vi "VIH UI - Project XML Indicator.vi"(11 "XML in":string) -> ()   [LabVIEW 2014]
doc: "::: VI Helpeks :::\nCopyright (c) 2000-2026 Konstantin Shifershteyn. All rights reserved."
panel:
  out "XML":string
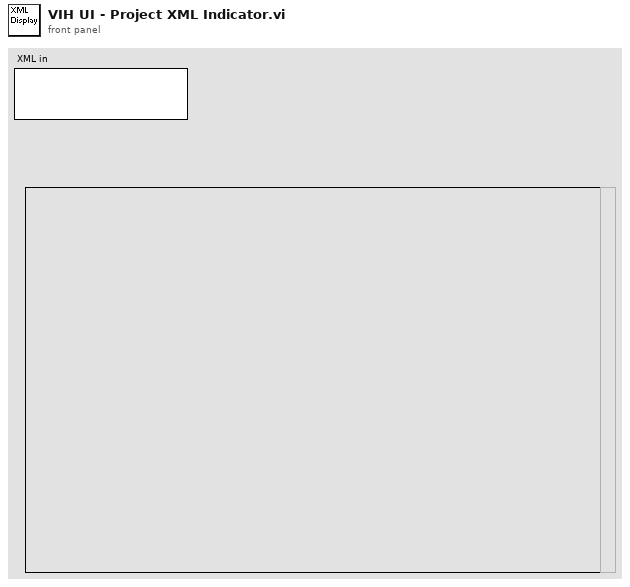
[diagram p1: front panel]
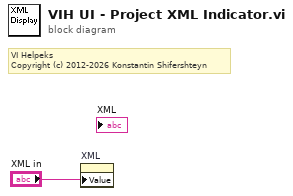
[diagram p0: block diagram]
diagram:
  # "VI Helpeks\nCopyright (c) 2012-2026 Konstantin Shifershteyn"
  n1 = property on="XML" class="Str"("Value"="XML in") -> ()  [unwired: 2 in, 2 out]
